vi "Order tree.vi"(7 "Tags map":refnum<vi>, 8 "error in":errorcluster, 11 "TreeControl in":refnum<vi>) -> (0 "error out":errorcluster)   [LabVIEW 2025, in "CAN-LIN Raw Bus Capture UI.lvlib"]
uses:
  CAN-LIN Raw Bus Capture UI.lvlib
  <vilib>/Array/Sort 2D Array - Pop Stack.vi
  <vilib>/Array/Sort 2D Array - Push Stack.vi
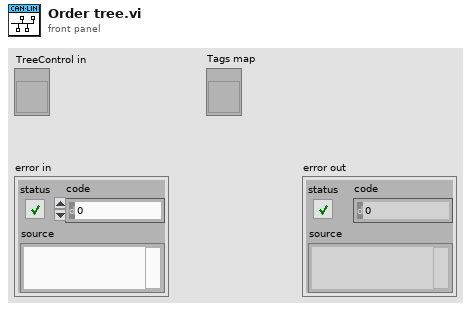
[diagram p1: front panel]
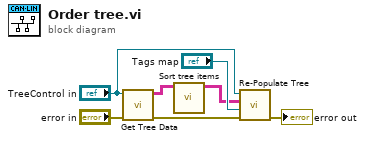
[diagram p0: block diagram]
diagram:
  n1 = call "Get Tree Data.vi"("error in"="error in", "Tree ref"="TreeControl in") -> ("error out"=w6:errorcluster, "Array"=w1:string[][])  [unwired: 8 in]
  n2 = call "Sort tree items.vi"("Array"=w1) -> ("sorted 2D array"=w2:string[][])  [unwired: 10 in]
  n3 = call "Re-Populate Tree.vi"("error in"=w6, "Tags map"="Tags map", "Data in"=w2, "TreeControl in"="TreeControl in") -> ("error out"=→"error out":errorcluster)  [unwired: 7 in]
